vi "ALL - CSE VIs.vi"() -> ()   [LabVIEW 2021]
doc: "::: CalcExpress Toolkit :::\nCopyright (c) 2000-2026 Konstantin Shifershteyn. All rights reserved."
uses:
  cetypes.llb/VarMan Variable Context Handle.ctl
  cse.llb/CSE Instance RefNum.ctl
  cse.llb/CSE Callback VI RefNum.ctl
  cse.llb/CSE Type - Run Mode.ctl
  cse.llb/CSE Type - Callback Call Reason.ctl
panel:
  in  "False":bool
  out "Stop/Call Reason":T1=1 items=["Exec Start", "Action completed", "pause to breath", "reserved 1", "reserved 2", "custom"]
  in  "CSE Run mode":T2 items=["Execute", "Abort", "Run", "Step", "Step Over", "Step Out", "Run (LM)", "Step (LM)", "Step Over (LM)", "Step Out (LM)", "unsupported"]
  in  "Callback VI RefNum":T3
  in  "CSE RefNum":T4
  in  "VC Handle":T5=-1
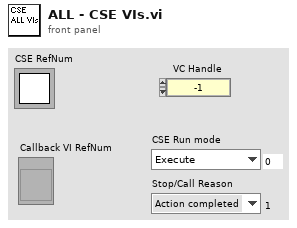
[diagram p1: front panel]
types:
  T1 = typedef "CSE Type - Callback Call Reason.ctl" = u32
  T2 = typedef "CSE Type - Run Mode.ctl" = u32
  T3 = typedef "CSE Callback VI RefNum.ctl" = refnum<vi>
  T4 = typedef "CSE Instance RefNum.ctl" = refnum<k1>
  T5 = typedef "VarMan Variable Context Handle.ctl" = i32
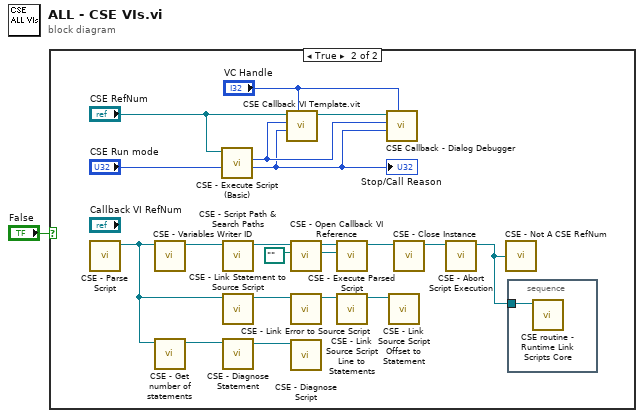
[diagram p0: block diagram]
diagram:
  n1 = case shown="True" "False" {
    frame False {
    }
    frame True {
      n2 = call "CSE - Parse Script.vi"() -> ("CSE RefNum"=w4:T4)  [unwired: 7 in, 4 out]
      n3 = call "CSE - Variables Writer ID.vi"("CSE RefNum"=w4) -> ("dup CSE RefNum"=w3:T4)  [unwired: 8 in, 2 out]
      n4 = call "CSE - Get number of statements.vi"("CSE RefNum"=w4) -> ("dup CSE RefNum"=w5:T4)  [unwired: 7 in, 3 out]
      n5 = call "CSE - Execute Script (Basic).vi"("Run mode"="CSE Run mode", "CSE RefNum"="CSE RefNum") -> ("Stop Reason"=w13:T1, "Stm Index out"=w14:i32)  [unwired: 5 in, 3 out]
      "Stop/Call Reason" <- w13
      n6 = call "CSE - Script Path & Search Paths.vi"("CSE RefNum"=w3) -> ("dup CSE RefNum"=w2:T4)  [unwired: 7 in, 3 out]
      n7 = call "CSE - Link Statement to Source Script.vi"("CSE RefNum"=w4) -> ("dup CSE RefNum"=w19:T4)  [unwired: 5 in, 5 out]
      n8 = call "CSE - Diagnose Statement.vi"("CSE RefNum"=w5) -> ("dup CSE RefNum"=w10:T4)  [unwired: 5 in, 5 out]
      n9 = call "CSE Callback VI Template.vit"("VC Handle"="VC Handle", "Call Reason"=w13, "Stm Index"=w14, "CSE RefNum"="CSE RefNum") -> ("dup CSE RefNum"=w16:T4)  [unwired: 2 in, 5 out]
      n10 = call "CSE - Open Callback VI Reference.vi"("Callback VI Path"=path "", "CSE RefNum"=w2) -> ("Callback VI RefNum"=w8:T3, "dup CSE RefNum"=w9:T4)  [unwired: 7 in, 1 out]
      n11 = call "CSE - Link Error to Source Script.vi"("CSE RefNum"=w19) -> ("dup CSE RefNum"=w18:T4)  [unwired: 4 in, 6 out]
      n12 = call "CSE - Diagnose Script.vi"("CSE RefNum"=w10) -> ()  [unwired: 8 in, 3 out]
      n13 = call "CSE - Execute Parsed Script.vi"("Callback VI RefNum"=w8, "CSE RefNum"=w9) -> ("dup CSE RefNum"=w21:T4)  [unwired: 5 in, 4 out]
      n14 = call "CSE - Link Source Script Line to Statements.vi"("CSE RefNum"=w18) -> ("dup CSE RefNum"=w11:T4)  [unwired: 7 in, 3 out]
      n15 = call "CSE Callback - Dialog Debugger.vi"("VC Handle"="VC Handle", "Call Reason"=w13, "Stm Index"=w14, "CSE RefNum"=w16) -> ()  [unwired: 2 in, 6 out]
      n16 = call "CSE - Link Source Script Offset to Statement.vi"("CSE RefNum"=w11) -> ()  [unwired: 7 in, 4 out]
      n17 = call "CSE - Close Instance.vi"("CSE RefNum"=w21) -> ("dup CSE RefNum"=w20:T4)  [unwired: 6 in, 2 out]
      n18 = call "CSE - Abort Script Execution.vi"("CSE RefNum"=w20) -> ("dup CSE RefNum"=w6:T4)  [unwired: 6 in, 2 out]
      n19 = call "CSE - Not A CSE RefNum.vi"("CSE RefNum"=w6) -> ()  [unwired: 2 out]
      n20 = stacked-sequence {
        tunnel: w6 -> [w22]
        frame #0 {
          n21 = call "CSE routine - Runtime Link Scripts Core.vi"("CSE RefNum"=w22) -> ()  [unwired: 5 in, 6 out]
        }
      }
    }
  }
